vi "Entry.vi"(8 "error in (no error)":errorcluster, 11 "New State":refnum<class "Manual.lvclass">) -> (0 "error out":errorcluster, 3 "State out":refnum<class "Manual.lvclass">)   [LabVIEW 2014, in "States.lvlib" / "Manual.lvclass"]
doc: "This is an abstract method. Override this method to define the behavior when you enter the state."
uses:
  Manual.lvclass
  ctl/P3AT_Current.ctl
  <vilib>/ActorFramework/Message Enqueuer/Message Enqueuer.lvclass/Message Enqueuer.ctl
  <vilib>/ActorFramework/Message Enqueuer/Enqueue.vi
  Global_var/Global_var.vi
  <vilib>/ActorFramework/Message Priority Queue/Priority Enqueue.vi
  Process State/CoordinatorState.lvclass
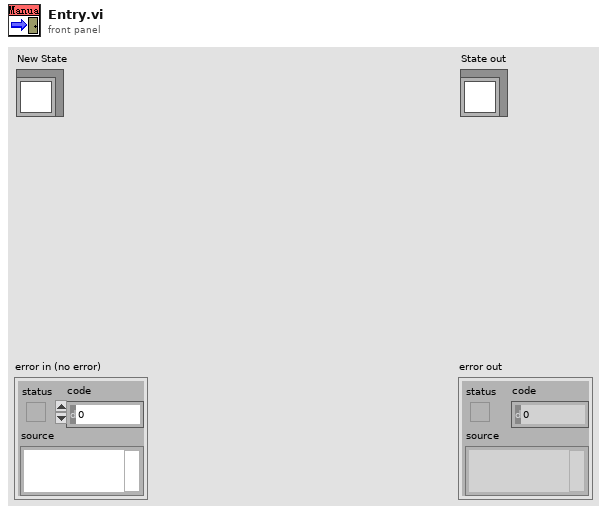
[diagram p1: front panel]
types:
  T1 = enum32{"Joy", "Map", "Voice", "Input", "Undefined"}
  T2 = typedef "P3AT_Current.ctl" = cluster{"max_vel":dbl, "max_rot":dbl, "now_pose_X":dbl, "now_pose_Y":dbl, "now_pose_Rot_deg":dbl, "Control_Mode":enum32{"Joy", "Map", "Voice", "Input", "Undefined"}}
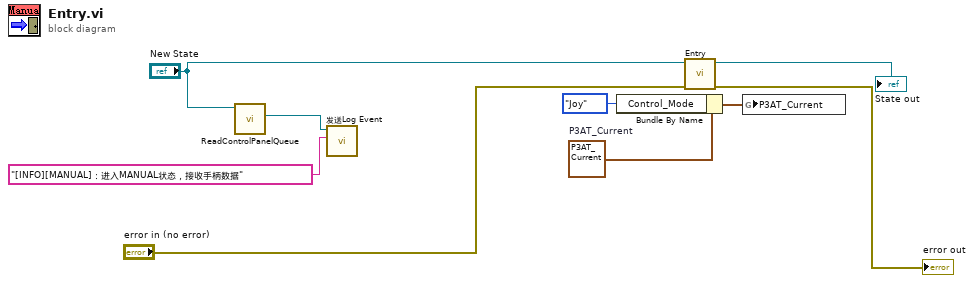
[diagram p0: block diagram]
diagram:
  w6 = T2 {"max_vel"=0.49056603773584906, "max_rot"=0.5094339622641509, "now_pose_X"=0.0, "now_pose_Y"=0.0, "now_pose_Rot_deg"=0.0, "Control_Mode"=enum."Joy"}  # P3AT_Current
  n1 = call-dynamic "ReadControlPanelQueue.vi"("CoordinatorState输入"="New State") -> ("操作者框架:消息待入队列"=w2:refnum<class "Message Enqueuer.lvclass">)  [unwired: 8 in, 2 out]
  n2 = call "发送Log Event.vi"("Event Text"="[INFO][MANUAL]：进入MANUAL状态，接收手柄数据", "消息待入队列"=w2) -> ()  [unwired: 8 in, 2 out]
  n3 = Bundle By Name(cluster=w6, "Control_Mode"=T1."Joy") -> (w5:T2)
  n4 = call-parent "Entry.vi"("error in (no error)"="error in (no error)", "New State"="New State") -> ("error out"=→"error out":errorcluster, "State out"=→"State out":refnum<class "Manual.lvclass">)  [unwired: 8 in]
  n5 = global write "Global_var.vi" "P3AT_Current"(w5) -> ()
